vi "Start Idle Processes if Running.vi"(8 "error in (no error)":errorcluster, 10 "Rig Process":refnum<class "Process.lvclass">, 11 "Application In":refnum<class "Application.lvclass">) -> (0 "error out":errorcluster, 2 "Rig Process Out":refnum<class "Process.lvclass">, 3 "Application Out":refnum<class "Application.lvclass">)   [LabVIEW 2020]
uses:
  Process/Process.lvclass
  Application.lvclass
  Process/Process.lvclass/Process.ctl
  <vilib>/Utility/error.llb/Clear Errors.vi
  Application.lvclass/Application.ctl
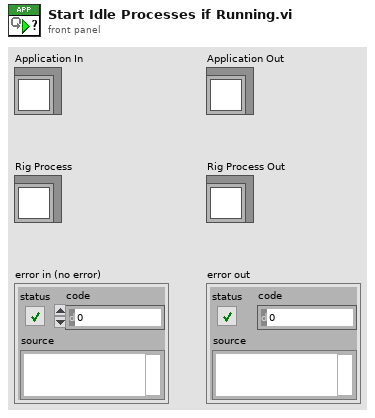
[diagram p1: front panel]
types:
  T1 = typedef "Process.lvclass/Lifecycle State.ctl" = enum16{"Uninitialized", "Initialized", "Started", "Running", "Stopped", "Finished"}
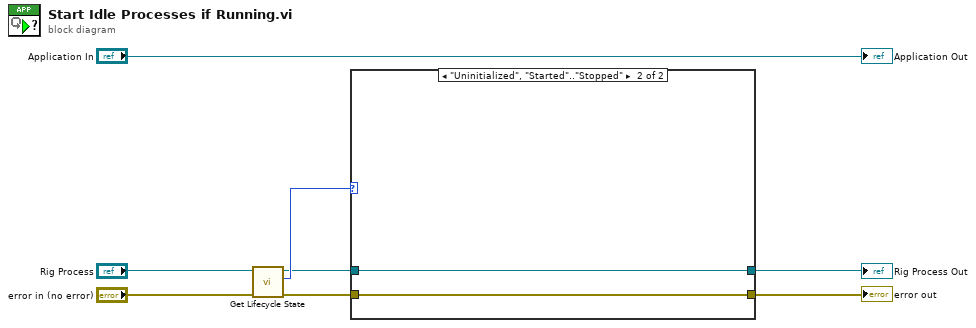
[diagram p0: block diagram]
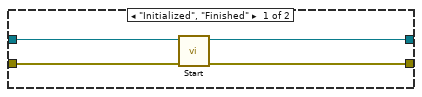
[diagram p2: hidden frame]
diagram:
  n1 = call "Get Lifecycle State.vi"("error in (no error)"="error in (no error)", "Process In"="Rig Process") -> ("error out"=w1:errorcluster, "Lifecycle State"=w3:T1, "Process Out"=w2:refnum<class "Process.lvclass">)  [unwired: 6 in, 1 out]
  n2 = case shown="\"Uninitialized\", \"Started\"..\"Stopped\"" w3 {
    tunnel: w2 -> [w12 w14]
    tunnel: w1 -> [w11 w13]
    tunnel: [w10 w13] -> w8
    tunnel: [w9 w14] -> w7
    frame "Initialized", "Finished" {
      n3 = call "Start.vi"("error in (no error)"=w11, "Process In"=w12) -> ("error out"=w10:errorcluster, "Process Out"=w9:refnum<class "Process.lvclass">)  [unwired: 7 in, 1 out]
    }
    frame "Uninitialized", "Started".."Stopped" {
    }
  }
  "error out" <- w8
  "Rig Process Out" <- w7
  "Application Out" <- "Application In"
